vi "Configuration Parse.vi"(0 "Measurement Configuration":T6={"Automation Test"=FALSE, "Power sequencing file path"="", "RFSG name"="5842", "RFSG port"="port1", "RFSG attenuation mode"=enum."<None>", "RFSG external attenuation (dB)"=2.0, "RFSG s-parameters orientation"=enum."Port1 Towards DUT", "RFSG s2p file path"="", "RFmx name"="5842", "RFmx port"="port2", "RFmx attenuation mode"=enum."<None>", "RFmx external attenuation (dB)"=7.0, "RFmx s-parameters orientation"=enum."Port1 Towards DUT", "RFmx s2p file path"="", "RFmx Center Frequency (Hz)"=10000000000.0, "RFmx Measurement Bandwidth (Hz)"=80000000.0, "RFmx Reference Level (dBm)"=10.0, "RFSG Generation IQ Rate (S/s)"=1250000000.0, "Pulse Acquisition Length (s)"=0.002, "Pulse Power Level (dBm)"=-20.0, "Pulse Repetition Interval [PRI] (s)"=0.0001, "Pulse Width (s)"=2e-05, "Number of Pulses per Burst"=20, "Measurement Offset"=0, "Window Start (%)"=10.0, "Window Stop (%)"=90.0, "Window Step Size (%)"=10.0, "High Reference Level (%)"=90.0, "Width Reference Level (%)"=50.0, "Low Reference Level (%)"=10.0, "Selected Pulse Trace"=0, "Power sequecing file validity check"=FALSE} {"High Reference Level (%)" min=0.0 max=100.0 step=1.0; "Low Reference Level (%)" min=0.0 max=100.0 step=1.0; "Width Reference Level (%)" min=0.0 max=100.0 step=1.0; "Window Step Size (%)" min=0.0 max=100.0 step=1.0; "Window Stop (%)" min=0.0 max=100.0 step=1.0; "Window Start (%)" min=0.0 max=100.0 step=1.0; "Pulse Acquisition Length (s)" format="%.2p"; "Pulse Width (s)" format="%#_6p"; "Pulse Repetition Interval [PRI] (s)" format="%#_6p"; "RFSG Generation IQ Rate (S/s)" format="%#_6p"; "RFmx Reference Level (dBm)" format="%.2f"; "RFmx Measurement Bandwidth (Hz)" format="%.3p"; "RFmx Center Frequency (Hz)" format="%.6p"; "RFmx external attenuation (dB)" format="%.2f"; "RFSG external attenuation (dB)" format="%.2f"}, 11 "error in":errorcluster) -> (4 "RFmx Settings":T1={"Center Frequency (Hz)"=10000000000.0, "Measurement Bandwidth (Hz)"=80000000.0, "Reference Level (dBm)"=10.0, "RFmx De-embedding"={"RFmx Name"="5842_0", "RFmx Port"="", "Attenuation"={"Mode"=enum."Constant Attenuation", "Constant Attenuation"={"RFmx External Attenuation (dB)"=1.2}, "s2p File"={"RFmx S-Parameters Orientation"=24000, "RFmx Attenuation s2p Path Name"="", "RFmx Attenuation s2p File"=path ""}}}, "Acquisition Length (s)"=0.0} {"RFmx De-embedding"."Attenuation"."s2p File"."RFmx S-Parameters Orientation" items=["Port1 Towards DUT"=24000, "Port2 Towards DUT"=24001]; "RFmx De-embedding"."Attenuation"."Constant Attenuation"."RFmx External Attenuation (dB)" format="%.2f"; "Reference Level (dBm)" format="%.2f"; "Measurement Bandwidth (Hz)" format="%.3p"; "Center Frequency (Hz)" format="%.6p"}, 6 "RFSG settings":T3={"RFSG De-embedding"={"RFSG Name"="5842_0", "RFSG Port"="", "Attenuation"={"Mode"=enum."Constant Attenuation", "Contant Attenuation"={"RFSG External Attenuation (dB)"=2.0}, "s2p File"={"RFSG S-parameters Orientation"=24000, "RFSG Attenuation s2p Path Name"="", "RFSG s2p File Path"=path ""}}}, "Generation IQ Rate (S/s)"=0.0} {"RFSG De-embedding"."Attenuation"."s2p File"."RFSG S-parameters Orientation" items=["Port1 Towards DUT"=24000, "Port2 Towards DUT"=24001]; "RFSG De-embedding"."Attenuation"."Contant Attenuation"."RFSG External Attenuation (dB)" format="%.2f"}, 8 "Test Configuration":T5, 15 "error out":errorcluster)   [LabVIEW 2023, in "FPT Pulse Measurement.lvclass"]
uses:
  FPT Pulse Measurement.lvclass
  Measurement Configuration.ctl
  Measurement/Controls/Test Config - Pulse.ctl
  Measurement/Controls/RFSG Config - Pulse.ctl
  FPT Shared VIs/De-embedding/RFsg Config.ctl
  Measurement/Controls/RFmx Config - Pulse.ctl
  FPT Shared VIs/De-embedding/RFmx Config.ctl
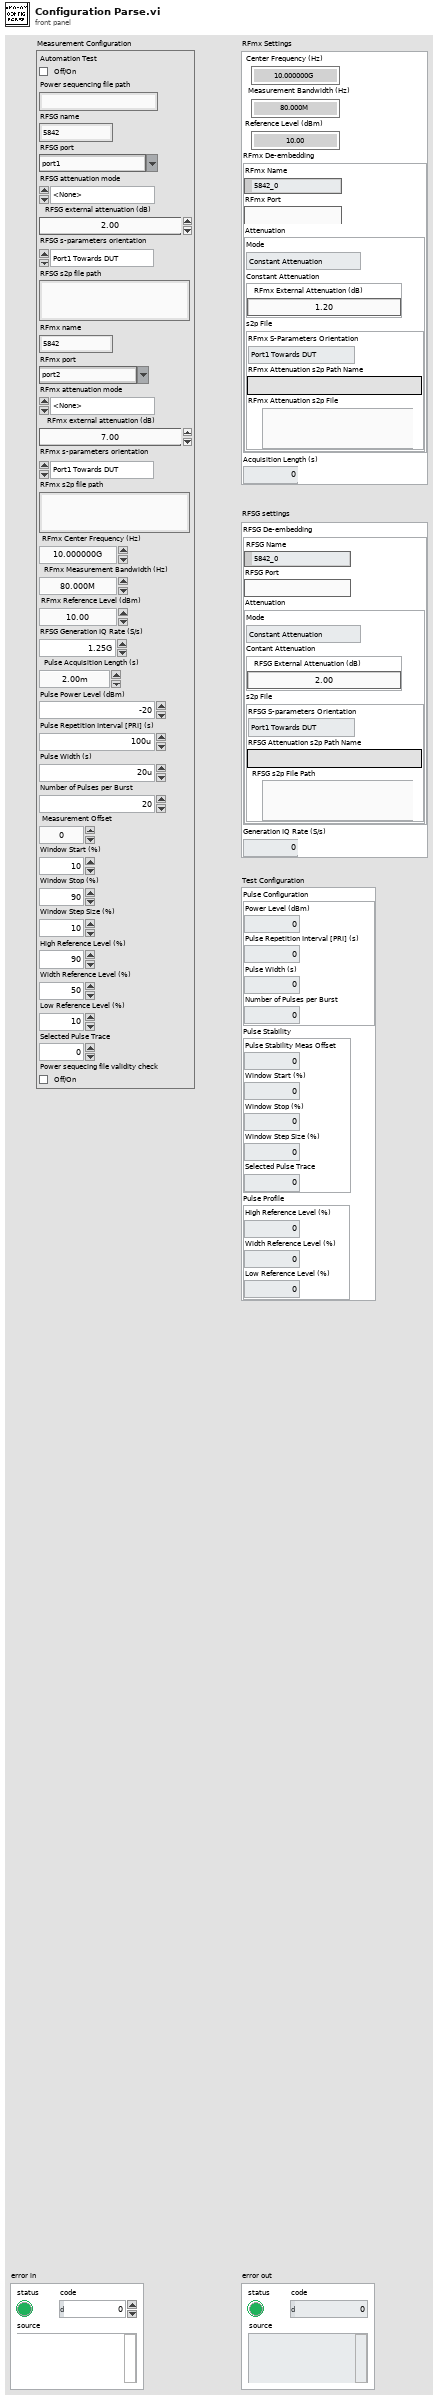
[diagram p1: front panel]
types:
  T1 = typedef "RFmx Config - Pulse.ctl" = cluster{"Center Frequency (Hz)":dbl, "Measurement Bandwidth (Hz)":dbl, "Reference Level (dBm)":dbl, "RFmx De-embedding":T2, "Acquisition Length (s)":dbl}
  T2 = typedef "RFmx Config.ctl" = cluster{"RFmx Name":refnum<k15>, "RFmx Port":string, "Attenuation":cluster{"Mode":enum32{"<None>", "Constant Attenuation", "s2p File"}, "Constant Attenuation":cluster{"RFmx External Attenuation (dB)":dbl}, "s2p File":cluster{"RFmx S-Parameters Orientation":i32, "RFmx Attenuation s2p Path Name":string, "RFmx Attenuation s2p File":path}}}
  T3 = typedef "RFSG Config - Pulse.ctl" = cluster{"RFSG De-embedding":T4, "Generation IQ Rate (S/s)":dbl}
  T4 = typedef "RFsg Config.ctl" = cluster{"RFSG Name":refnum<k15>, "RFSG Port":string, "Attenuation":cluster{"Mode":enum32{"<None>", "Constant Attenuation", "s2p File"}, "Contant Attenuation":cluster{"RFSG External Attenuation (dB)":dbl}, "s2p File":cluster{"RFSG S-parameters Orientation":i32, "RFSG Attenuation s2p Path Name":string, "RFSG s2p File Path":path}}}
  T5 = typedef "Test Config - Pulse.ctl" = cluster{"Pulse Configuration":cluster{"Power Level (dBm)":dbl, "Pulse Repetition Interval [PRI] (s)":dbl, "Pulse Width (s)":dbl, "Number of Pulses per Burst":u32}, "Pulse Stability":cluster{"Pulse Stability Meas Offset":i32, "Window Start (%)":dbl, "Window Stop (%)":dbl, "Window Step Size (%)":dbl, "Selected Pulse Trace":i32}, "Pulse Profile":cluster{"High Reference Level (%)":dbl, "Width Reference Level (%)":dbl, "Low Reference Level (%)":dbl}}
  T6 = typedef "FPT Pulse Measurement.lvclass/Measurement Configuration.ctl" = cluster{"Automation Test":bool, "Power sequencing file path":string, "RFSG name":string, "RFSG port":string, "RFSG attenuation mode":enum32{"<None>", "Constant Attenuation", "s2p File"}, "RFSG external attenuation (dB)":dbl, "RFSG s-parameters orientation":enum32{"Port1 Towards DUT", "Port2 Towards DUT"}, "RFSG s2p file path":string, "RFmx name":string, "RFmx port":string, "RFmx attenuation mode":enum32{"<None>", "Constant Attenuation", "s2p File"}, "RFmx external attenuation (dB)":dbl, "RFmx s-parameters orientation":enum32{"Port1 Towards DUT", "Port2 Towards DUT"}, "RFmx s2p file path":string, "RFmx Center Frequency (Hz)":dbl, "RFmx Measurement Bandwidth (Hz)":dbl, "RFmx Reference Level (dBm)":dbl, "RFSG Generation IQ Rate (S/s)":dbl, "Pulse Acquisition Length (s)":dbl, "Pulse Power Level (dBm)":dbl, "Pulse Repetition Interval [PRI] (s)":dbl, "Pulse Width (s)":dbl, "Number of Pulses per Burst":u32, "Measurement Offset":i32, "Window Start (%)":dbl, "Window Stop (%)":dbl, "Window Step Size (%)":dbl, "High Reference Level (%)":dbl, "Width Reference Level (%)":dbl, "Low Reference Level (%)":dbl, "Selected Pulse Trace":i32, "Power sequecing file validity check":bool}
  T7 = enum32{"<None>", "Constant Attenuation", "s2p File"}
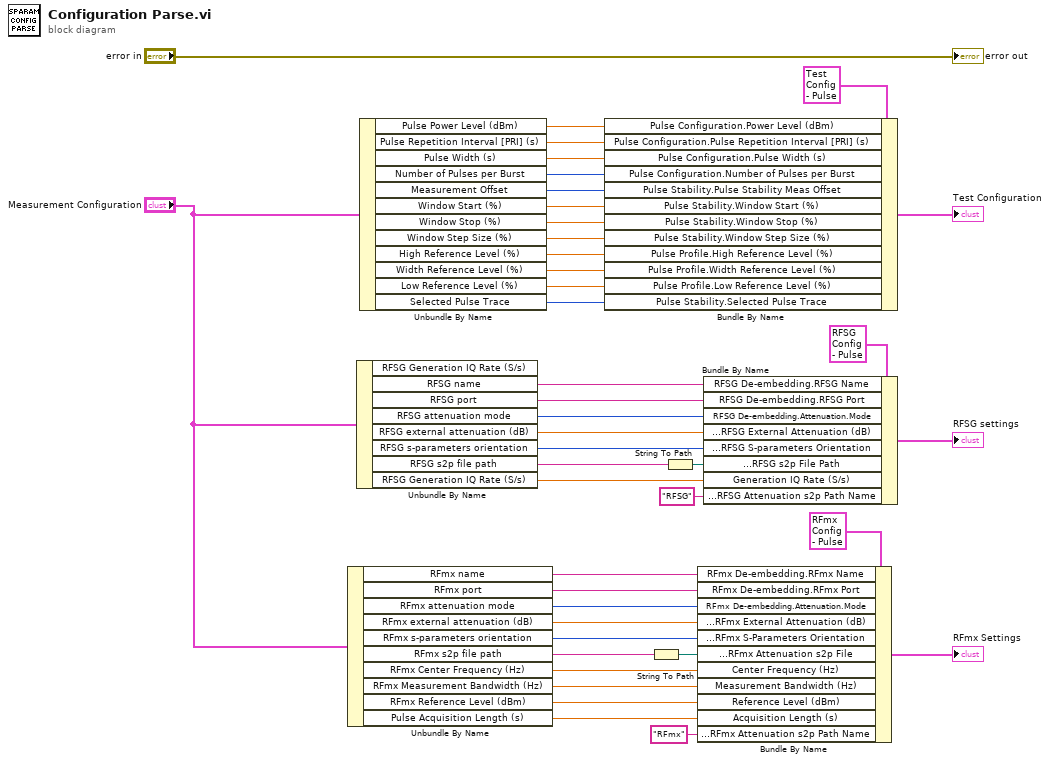
[diagram p0: block diagram]
diagram:
  n1 = Unbundle By Name("Measurement Configuration") -> ("RFmx name"=w18:string, "RFmx port"=w19:string, "RFmx attenuation mode"=w24:T7, "RFmx external attenuation (dB)"=w23:dbl, "RFmx s-parameters orientation"=w22:enum32{"Port1 Towards DUT", "Port2 Towards DUT"}, "RFmx s2p file path"=w20:string, "RFmx Center Frequency (Hz)"=w8:dbl, "RFmx Measurement Bandwidth (Hz)"=w7:dbl, "RFmx Reference Level (dBm)"=w6:dbl, "Pulse Acquisition Length (s)"=w5:dbl)
  n2 = Unbundle By Name("Measurement Configuration") -> ("RFSG name"=w16:string, "RFSG port"=w15:string, "RFSG attenuation mode"=w29:T7, "RFSG external attenuation (dB)"=w28:dbl, "RFSG s-parameters orientation"=w27:enum32{"Port1 Towards DUT", "Port2 Towards DUT"}, "RFSG s2p file path"=w26:string, "RFSG Generation IQ Rate (S/s)"=w11:dbl)  [unwired: 1 out]
  n3 = Unbundle By Name("Measurement Configuration") -> ("Pulse Power Level (dBm)"=w40:dbl, "Pulse Repetition Interval [PRI] (s)"=w39:dbl, "Pulse Width (s)"=w38:dbl, "Number of Pulses per Burst"=w37:u32, "Measurement Offset"=w36:i32, "Window Start (%)"=w35:dbl, "Window Stop (%)"=w34:dbl, "Window Step Size (%)"=w33:dbl, "High Reference Level (%)"=w32:dbl, "Width Reference Level (%)"=w31:dbl, "Low Reference Level (%)"=w30:dbl, "Selected Pulse Trace"=w1:i32)
  n4 = Bundle By Name(cluster=T5 {"Pulse Configuration"={"Power Level (dBm)"=0.0, "Pulse Repetition Interval [PRI] (s)"=0.0, "Pulse Width (s)"=0.0, "Number of Pulses per Burst"=0}, "Pulse Stability"={"Pulse Stability Meas Offset"=0, "Window Start (%)"=0.0, "Window Stop (%)"=0.0, "Window Step Size (%)"=0.0, "Selected Pulse Trace"=0}, "Pulse Profile"={"High Reference Level (%)"=0.0, "Width Reference Level (%)"=0.0, "Low Reference Level (%)"=0.0}} ("Test Configuration"), "Pulse Configuration.Power Level (dBm)"=w40, "Pulse Configuration.Pulse Repetition Interval [PRI] (s)"=w39, "Pulse Configuration.Pulse Width (s)"=w38, "Pulse Configuration.Number of Pulses per Burst"=w37, "Pulse Stability.Pulse Stability Meas Offset"=w36, "Pulse Stability.Window Start (%)"=w35, "Pulse Stability.Window Stop (%)"=w34, "Pulse Stability.Window Step Size (%)"=w33, "Pulse Profile.High Reference Level (%)"=w32, "Pulse Profile.Width Reference Level (%)"=w31, "Pulse Profile.Low Reference Level (%)"=w30, "Pulse Stability.Selected Pulse Trace"=w1) -> (→"Test Configuration":T5)
  n5 = String To Path(string=w20) -> (path=w21:path)
  n6 = String To Path(string=w26) -> (path=w25:path)
  n7 = Bundle By Name(cluster=T1 {"Center Frequency (Hz)"=10000000000.0, "Measurement Bandwidth (Hz)"=80000000.0, "Reference Level (dBm)"=10.0, "RFmx De-embedding"={"RFmx Name"="5842_0", "RFmx Port"="", "Attenuation"={"Mode"=enum."Constant Attenuation", "Constant Attenuation"={"RFmx External Attenuation (dB)"=1.2}, "s2p File"={"RFmx S-Parameters Orientation"=24000, "RFmx Attenuation s2p Path Name"="", "RFmx Attenuation s2p File"=path ""}}}, "Acquisition Length (s)"=0.0} ("RFmx Settings"), "RFmx De-embedding.RFmx Name"=w18, "RFmx De-embedding.RFmx Port"=w19, "RFmx De-embedding.Attenuation.Mode"=w24, "RFmx De-embedding.Attenuation.Constant Attenuation.RFmx External Attenuation (dB)"=w23, "RFmx De-embedding.Attenuation.s2p File.RFmx S-Parameters Orientation"=w22, "RFmx De-embedding.Attenuation.s2p File.RFmx Attenuation s2p File"=w21, "Center Frequency (Hz)"=w8, "Measurement Bandwidth (Hz)"=w7, "Reference Level (dBm)"=w6, "Acquisition Length (s)"=w5, "RFmx De-embedding.Attenuation.s2p File.RFmx Attenuation s2p Path Name"="RFmx") -> (→"RFmx Settings":T1)
  n8 = Bundle By Name(cluster=T3 {"RFSG De-embedding"={"RFSG Name"="5842_0", "RFSG Port"="", "Attenuation"={"Mode"=enum."Constant Attenuation", "Contant Attenuation"={"RFSG External Attenuation (dB)"=2.0}, "s2p File"={"RFSG S-parameters Orientation"=24000, "RFSG Attenuation s2p Path Name"="", "RFSG s2p File Path"=path ""}}}, "Generation IQ Rate (S/s)"=0.0} ("RFSG settings"), "RFSG De-embedding.RFSG Name"=w16, "RFSG De-embedding.RFSG Port"=w15, "RFSG De-embedding.Attenuation.Mode"=w29, "RFSG De-embedding.Attenuation.Contant Attenuation.RFSG External Attenuation (dB)"=w28, "RFSG De-embedding.Attenuation.s2p File.RFSG S-parameters Orientation"=w27, "RFSG De-embedding.Attenuation.s2p File.RFSG s2p File Path"=w25, "Generation IQ Rate (S/s)"=w11, "RFSG De-embedding.Attenuation.s2p File.RFSG Attenuation s2p Path Name"="RFSG") -> (→"RFSG settings":T3)
  "error out" <- "error in"
